vi "Main.vi"(11 "Module Admin":refnum<class "Delacor_lib_QMH_Module Admin.lvclass">) -> ()   [LabVIEW 2026, in "Launcher.lvlib"]
doc: "This template is based off of the Queued Message Handler design pattern and the Queued Message Handler project template that ships with LabVIEW.\n\nThe main difference is that the queue is private to this module and communication between modules is performed via Broadcast and Request events.\n\nRequest events are wrapped in public API methods and are handled in the Event Handling Loop (EHL) of this VI. Any module can register for Broadcast events sent by this module. The EHL generates messages based on user interface actions.\n\nThe Message Handling Loop (MHL) processes messages generated by the EHL, or by other messages. The messages are string values, so new messages can be added easily to the Message Cases case structure in the MHL. Each message cluster can also provide an optional value for Message Data, which is a variant that can be converted to whatever message-specific data is required.\n_____\nBased on DQMH Dev Tools: Project Template 7.1.2.1547."
uses:
  Launcher.lvlib
  <vilib>/Delacor/Delacor QMH/Libraries/Module Admin_class/Delacor_lib_QMH_Module Admin.lvclass
  <vilib>/Wovalab/Utilities/Helper Loop Periodic Timing/Late Execution Mode--enum.ctl
  <vilib>/Wovalab/Utilities/Helper Loop Periodic Timing/Helper Loop Periodic Timing.lvclass/Helper Loop Periodic Timing.ctl
  Module Data--cluster.ctl
  Mode.ctl
  ReplayMode.ctl
  RecordMode.ctl
  Capture detection loop data--cluster.ctl
  <vilib>/Delacor/Delacor QMH/Libraries/Message Queue_class/Delacor_lib_QMH_Message Queue.lvclass/Delacor_lib_QMH_Message Queue.ctl
  Stop Argument--cluster.ctl
  <vilib>/Delacor/Delacor QMH/Libraries/Module Admin_class/Delacor_lib_QMH_Module Admin.lvclass/Delacor_lib_QMH_Module Admin.ctl
  Set Captures Folder Argument--cluster.ctl
  Set Capture Detection Loop Timeout Argument--cluster.ctl
  Trigger Capture Detection Loop Argument--cluster.ctl
  Trigger Capture Detection Loop (Reply Payload)--cluster.ctl
  Set Application Mode Argument--cluster.ctl
  Set Run ID to Replay Argument--cluster.ctl
  <vilib>/Utility/miscctls.llb/LVPointTypeDef.ctl
  <vilib>/Delacor/Delacor QMH/Libraries/Message Queue_class/Delacor_lib_QMH_Enqueue Message (Single).vi
  <vilib>/Delacor/Delacor QMH/Libraries/Module Admin_class/Delacor_lib_QMH_Get External Launch.vi
  <vilib>/Wovalab/Utilities/Helper Loop Periodic Timing/Stop Helper Loop Internal.vi
  <vilib>/Wovalab/Utilities/Helper Loop Periodic Timing/U32 Max Value--constant.vi
  <vilib>/Wovalab/Utilities/Helper Loop Periodic Timing/Update Last Execution Time.vi
  <vilib>/Wovalab/Utilities/Helper Loop Periodic Timing/Loops Events AE.vi
  <vilib>/Wovalab/Utilities/Helper Loop Periodic Timing/Notify Monitoring Window.vi
  <vilib>/Wovalab/Utilities/Helper Loop Periodic Timing/Monitoring--global.vi
  <vilib>/Wovalab/Utilities/Helper Loop Periodic Timing/Helper Loop Periodic Timing.lvclass
  <vilib>/Delacor/Delacor QMH/Libraries/Message Queue_class/Delacor_lib_QMH_Message Queue.lvclass
  UserEventRecorder/UserEventRecorder.lvlib
  Core/Core.lvlib
  replay/Replay/src/Libraries/Replay/Replay.lvlib
panel:
  out "error out":errorcluster
  out "Status":string
  in  "Simulate MHL Error":bool
  in  "Simulate EHL Error":bool
  # "Other processes communicate with this Module via its Public API (wrappers for its Request Events).\n\nThis Module communicates with other processes via its Broadcast Events.\nAny process that wants to receive these messages can register for this module's Broadcast events."
  # "This template is for the DQMH framework. See the block diagram for more information on how to use this template."
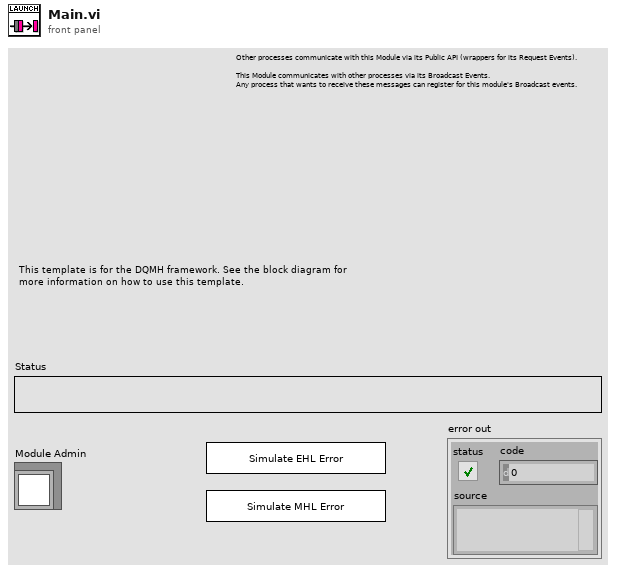
[diagram p1: front panel]
types:
  T1 = typedef "Wovalab_lib_Utilities.lvlib/Helper Loop Periodic Timing.lvclass/Late Execution Mode--enum.ctl" = enum16{"No change", "Process missed periods ignoring original phase", "Process missed periods maintaining original phase"}
  T2 = typedef "Launcher.lvlib/Broadcast Events--cluster.ctl" = cluster{"Module Did Init":refnum<user-event>, "Status Updated":refnum<user-event>, "Error Reported":refnum<user-event>, "Module Did Stop":refnum<user-event>, "Update Module Execution Status":refnum<user-event>, "Start Capture Detection Loop":refnum<user-event>, "Benchmark Started":refnum<user-event>, "Broadcast number of frames and run ID":refnum<user-event>}
  T3 = typedef "Launcher.lvlib/Request Events--cluster.ctl" = cluster{"Stop Module":refnum<user-event>, "Show Panel":refnum<user-event>, "Hide Panel":refnum<user-event>, "Get Module Execution Status":refnum<user-event>, "Show Diagram":refnum<user-event>, "Set Captures Folder":refnum<user-event>, "Set Capture Detection Loop Timeout":refnum<user-event>, "Trigger Capture Detection Loop":refnum<user-event>, "Set Application Mode":refnum<user-event>, "Application Mode":refnum<user-event>, "Set Run ID to Replay":refnum<user-event>, "Set Replay Run ID":refnum<user-event>}
  T4 = typedef "Capture detection loop data--cluster.ctl" = cluster{"Period":i32, "Reset":bool, "Iteration":i32, "Capture":path, "Mode":T5, "Replay Run ID":string, "Frame Number":u32, "Core Module ID":i32, "EventRecorderLaunched":bool, "Frame 0 relative seconds":dbl, "Record Run ID":string}
  T5 = typedef "Mode.ctl" = cluster{"Replay":T6, "Record":T7}
  T6 = typedef "ReplayMode.ctl" = enum16{"None", "User Events"}
  T7 = typedef "RecordMode.ctl" = enum16{"None", "User Events", "Benchmarks", "User Events and Benchmarks"}
  T8 = typedef "Launcher.lvlib/Module Data--cluster.ctl" = cluster{"Status":string, "Captures":path, "Capture Detection Loop Timeout":i32, "Mode":T5, "Replay Run ID":string, "Module Launched Timestamp":timestamp, "Record Run ID":i32, "Core Run ID":i32}
  T9 = enum32{"invalid lock state", "Not Locked", "Locked (No Password)", "Password-protected"}
  T10 = typedef "Launcher.lvlib/Stop Argument--cluster.ctl" = cluster{"Origin":string, "Exit via Stop Module Req?":bool, "Wait for Module to stop?":bool}
  T11 = typedef "Launcher.lvlib/Set Captures Folder Argument--cluster.ctl" = cluster{"Captures":path}
  T12 = typedef "Launcher.lvlib/Set Capture Detection Loop Timeout Argument--cluster.ctl" = cluster{"Timeout":i32}
  T13 = typedef "Launcher.lvlib/Trigger Capture Detection Loop Argument--cluster.ctl" = cluster{"Capture Detection Loop Timeout":i32, "Wait Notifier":refnum<notifier>, "wait for reply":bool}
  T14 = typedef "Launcher.lvlib/Set Application Mode Argument--cluster.ctl" = cluster{"Mode":T5}
  T15 = typedef "Launcher.lvlib/Set Run ID to Replay Argument--cluster.ctl" = cluster{"Run ID":string}
  T16 = typedef "LVPointTypeDef.ctl" = cluster{"Horizontal":i16, "Vertical":i16}
  T17 = enum32{"Invalid", "Standard", "Closed", "Hidden", "Minimized", "Maximized"}
  T18 = typedef "Launcher.lvlib/Trigger Capture Detection Loop (Reply Payload)--cluster.ctl" = cluster{"Module Initial Time Stamp":timestamp, "error":errorcluster}
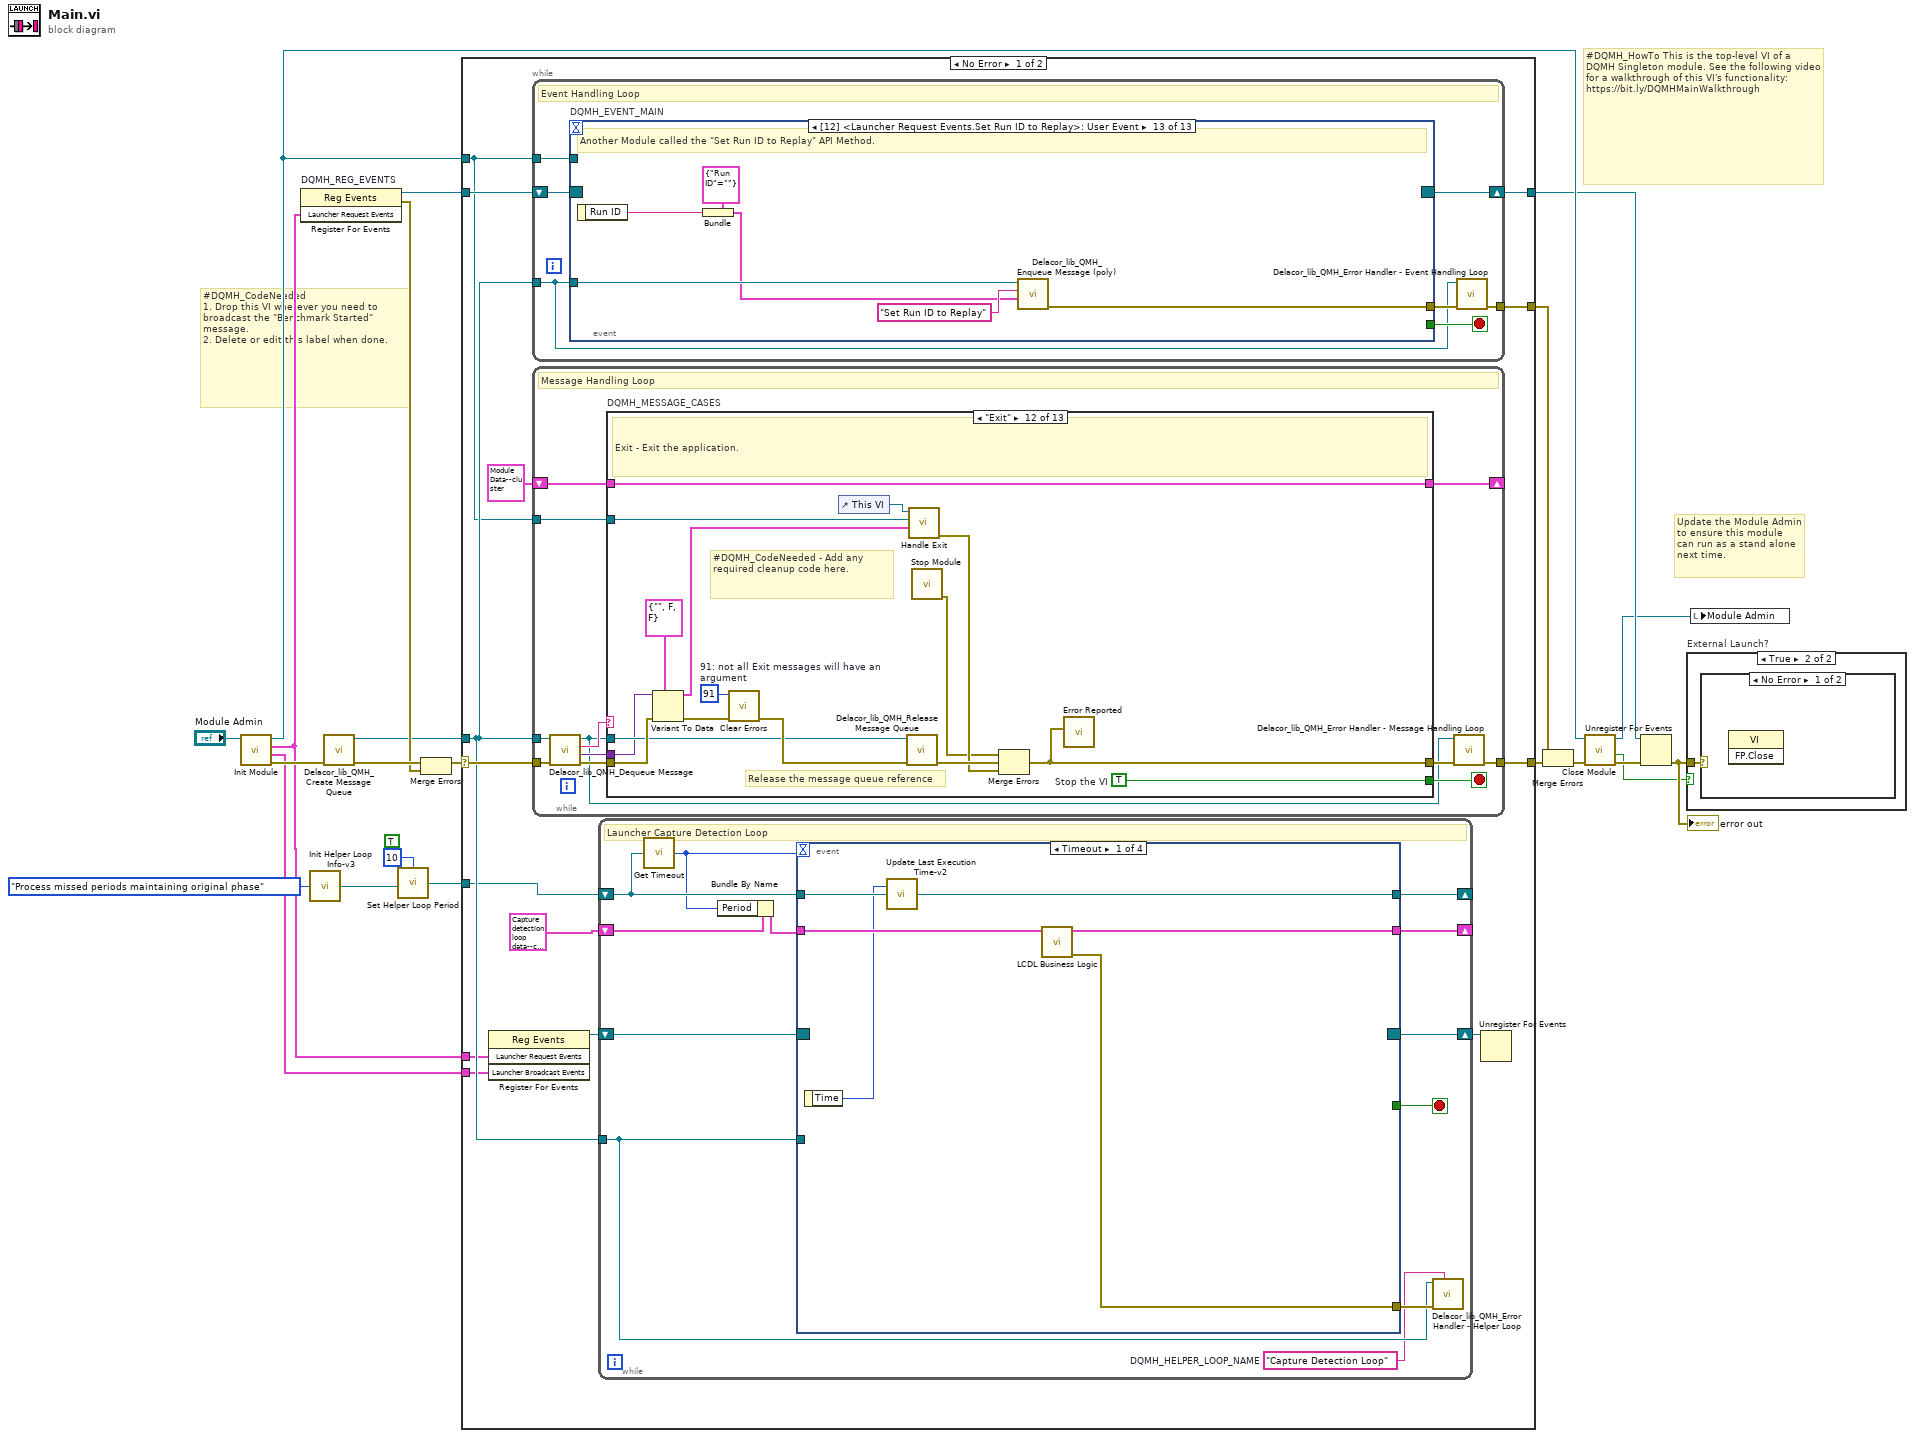
[diagram p0: block diagram]
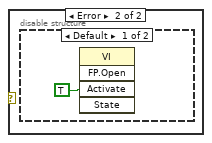
[diagram p3: hidden frame]
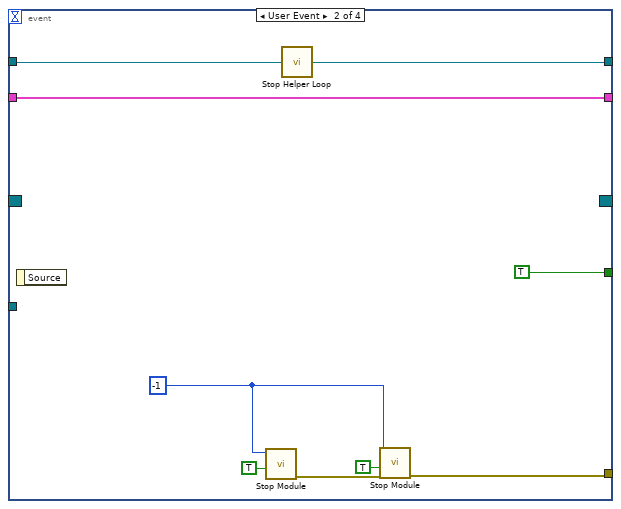
[diagram p5: hidden frame]
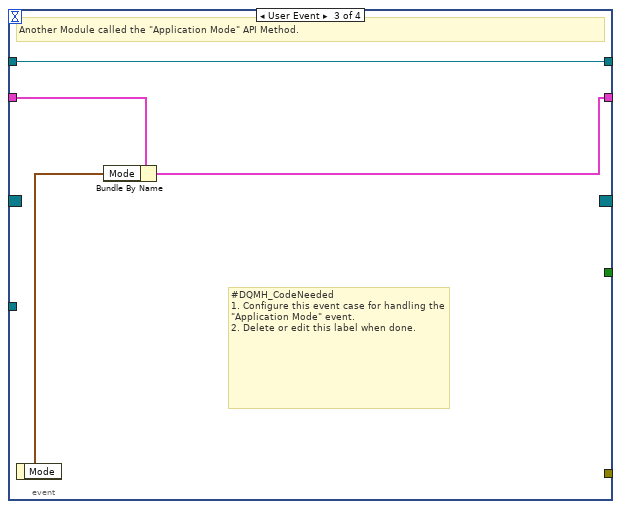
[diagram p6: hidden frame]
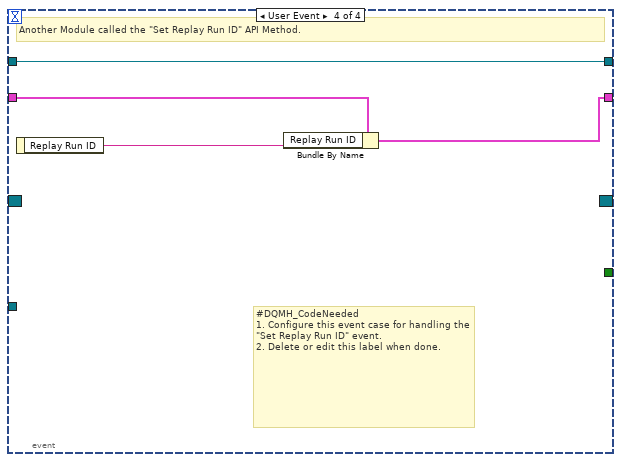
[diagram p7: hidden frame]
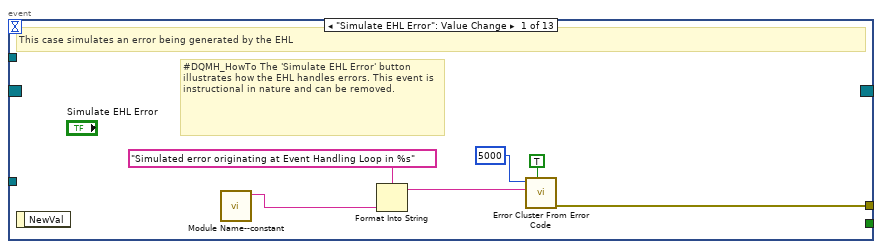
[diagram p8: hidden frame]
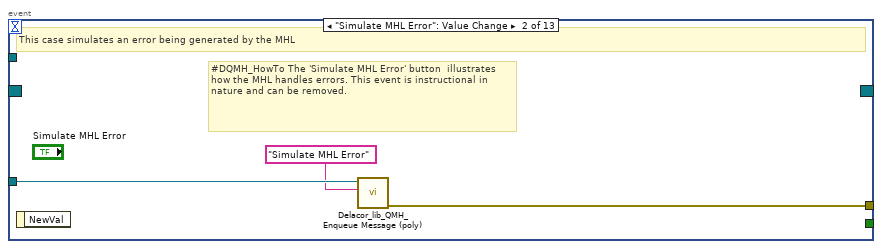
[diagram p9: hidden frame]
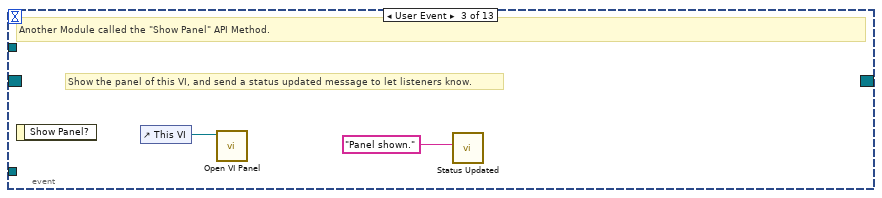
[diagram p10: hidden frame]
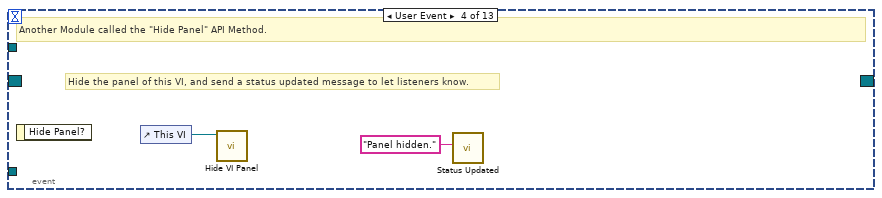
[diagram p11: hidden frame]
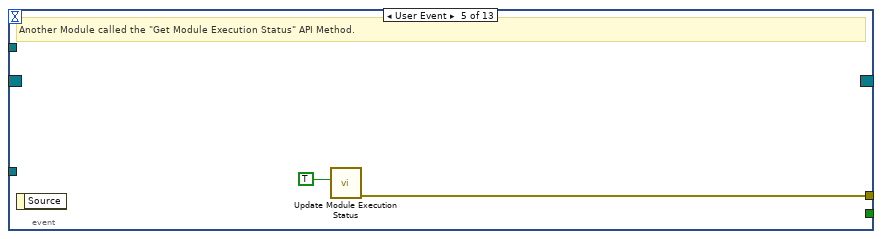
[diagram p12: hidden frame]
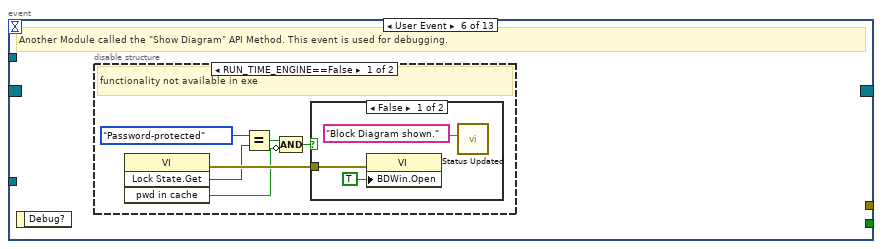
[diagram p13: hidden frame]
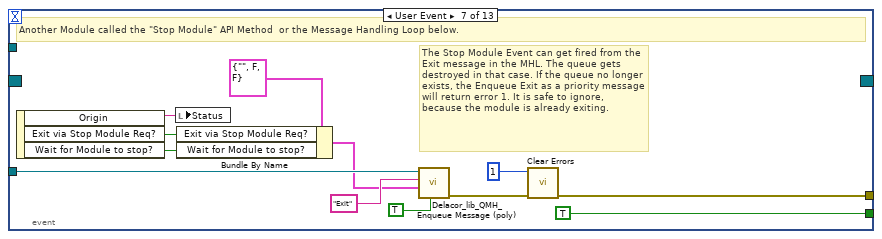
[diagram p16: hidden frame]
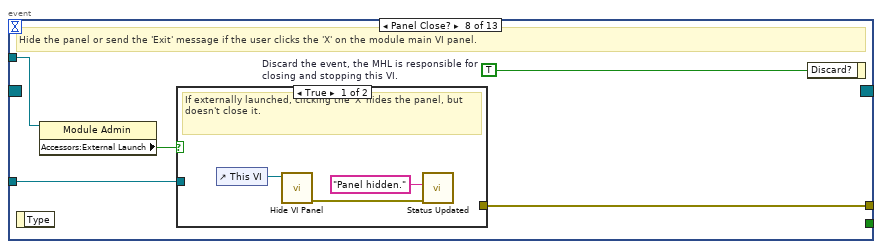
[diagram p17: hidden frame]
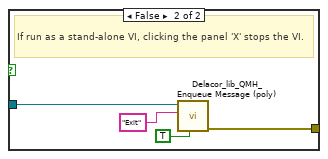
[diagram p18: hidden frame]
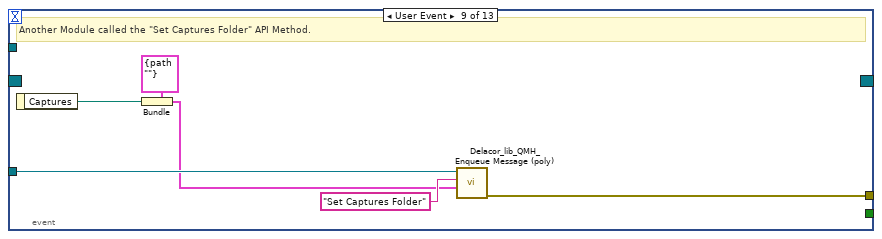
[diagram p19: hidden frame]
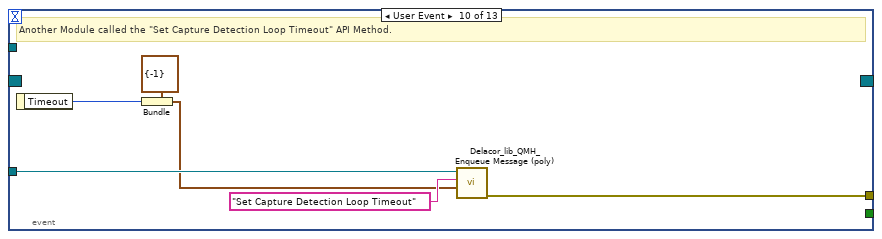
[diagram p20: hidden frame]
diagram:
  (unwired) TRUE ("Execute First Iteration ASAP (T)")
  # "#DQMH_CodeNeeded\n1. Drop this VI wherever you need to broadcast the \"Broadcast Latest Frame\" message.\n2. Delete or edit this label when done."
  # "#DQMH_CodeNeeded\n1. Drop this VI wherever you need to broadcast the \"Benchmark Started\" message.\n2. Delete or edit this label when done."
  # "#DQMH_HowTo This is the top-level VI of a DQMH Singleton module. See the following video for a walkthrough of this VI's functionality: https://bit.ly/DQMHMainWalkthrough"
  # "Update the Module Admin to ensure this module can run as a stand alone next time."
  n1 = call "Init Module.vi"("Singleton Module Admin in"="Module Admin") -> ("error out"=w21:errorcluster, "Launcher Broadcast Events"=w5:T2, "Launcher Request Events"=w6:T3, "Singleton Module Admin out"=w13:refnum<class "Delacor_lib_QMH_Module Admin.lvclass">)  [unwired: 7 in]
  n2 = register-events "DQMH_REG_EVENTS"(w6) -> (reference out=w11:refnum<event-registration>, error out=w14:errorcluster)  [unwired: 2 in]
  n3 = call <vilib>:"Init Helper Loop Info-v3.vi"("Late Execution Mode (Process missed periods ignoring original phase)"=Late_Execution_Mode--enum."Process missed periods maintaining original phase") -> ("Helper Loop Periodic Timing"=w3:refnum<class "Helper Loop Periodic Timing.lvclass">)  [unwired: 1 in]
  n4 = call <vilib>:"Delacor_lib_QMH_Create Message Queue.vi"("error in"=w21) -> ("error out"=w16:errorcluster, "Message Queue"=w10:refnum<class "Delacor_lib_QMH_Message Queue.lvclass">)  [unwired: 9 in]
  n5 = call <vilib>:"Set Helper Loop Period.vi"("Period (ms)"=10, "Helper Loop Periodic Timing in"=w3) -> ("Helper Loop Periodic Timing out"=w2:refnum<class "Helper Loop Periodic Timing.lvclass">)  [unwired: 13 in]
  n6 = Merge Errors(w16, w14) -> (w15:errorcluster)
  n7 = case shown="No Error" w15 {
    selector: w15 -> [w34 w321]
    tunnel: [w36 w320] -> w22
    tunnel: [w33 w319] -> w12
    tunnel: w11 -> [w31 w319]
    tunnel: w10 -> [w30 w314]
    tunnel: [w35 _] -> w19
    tunnel: w13 -> [w29 w315]
    tunnel: w6 -> [w28 _]
    tunnel: w5 -> [w25 _]
    tunnel: w2 -> [w23 _]
    frame No Error {
      n8 = register-events ("DQMH_HELPER_REGFOREVENTS")(w28, w25) -> (reference out=w26:refnum<event-registration>)  [unwired: 2 in, 1 out]
      n9 = while {
        tunnel: w30 -> [w72]
        shift-right: [w75] -> w33
        shift-left: w31 -> [w76]
        tunnel: [w77] -> w35
        tunnel: w29 -> [w73]
        stop <- w74 stop-if-true
        # "Event Handling Loop"
        n10 = event "DQMH_EVENT_MAIN" shown="[12] <Launcher Request Events.Set Run ID to Replay>: User Event" {
          selector: w76 -> [_ _ _ _ _ _ _ _ _ _ _ _ _]
          dyn-events: [_ _ _ _ _ _ _ _ _ _ _ _ _] -> w75
          timeout: _ -> [_ _ _ _ _ _ _ _ _ _ _ _ _]
          tunnel: [_ _ _ _ _ _ TRUE ("Discard?") _ _ _ _ _ _] -> w74
          tunnel: w72 -> [_ w86 _ _ _ _ w110 w117 w132 w138 w146 w152 w158]
          tunnel: [w84 w87 _ _ w93 _ w113 w119 w127 w133 w139 w147 w153] -> w78
          tunnel: w73 -> [_ _ _ _ _ _ _ w116 _ _ _ _ _]
          event "Simulate EHL Error": Value Change {
            # "#DQMH_HowTo The 'Simulate EHL Error' button  illustrates how the EHL handles errors. This event is instructional in nature and can be removed."
            # "This case simulates an error being generated by the EHL"
            n11 = event-data() -> ()  [unwired: 1 in, 1 out]
            n12 = call "Module Name--constant.vi"() -> ("Module Name"=w81:string)  [unwired: 11 in]
            n13 = Format Into String(format string="Simulated error originating at Event Handling Loop in %s", w81) -> (resulting string=w82:string)  [unwired: 2 in, 1 out]
            n14 = call <vilib>:"Error Cluster From Error Code.vi"("show call chain? (False)"=TRUE, "error message (\"\")"=w82, "error code (0)"=5000) -> ("error out"=w84:errorcluster)  [unwired: 6 in]
          }
          event "Simulate MHL Error": Value Change {
            # "#DQMH_HowTo The 'Simulate MHL Error' button  illustrates how the MHL handles errors. This event is instructional in nature and can be removed."
            # "This case simulates an error being generated by the MHL"
            n15 = event-data() -> ()  [unwired: 1 in, 1 out]
            n16 = call-poly <vilib>:"Delacor_lib_QMH_Enqueue Message (poly).vi"("Message"="Simulate MHL Error", "Message Queue in"=w86) -> ("error out"=w87:errorcluster)  [unwired: 8 in, 1 out]
          }
          event User Event {
            # "Show the panel of this VI, and send a status updated message to let listeners know."
            # "Another Module called the \"Show Panel\" API Method."
            n17 = event-data() -> ()  [unwired: 1 in, 1 out]
            n18 = control-ref of="This VI"() -> (w89:refnum<vi>)
            n19 = call "Open VI Panel.vi"("VI"=w89) -> ()  [unwired: 10 in, 1 out]
            n20 = call "Status Updated.vi"("Status"="Panel shown." ("format string")) -> ()  [unwired: 10 in, 1 out]
          }
          event User Event {
            # "Hide the panel of this VI, and send a status updated message to let listeners know."
            # "Another Module called the \"Hide Panel\" API Method."
            n21 = event-data() -> ()  [unwired: 1 in, 1 out]
            n22 = control-ref of="This VI"() -> (w91:refnum<vi>)
            n23 = call "Hide VI Panel.vi"("VI"=w91) -> ()  [unwired: 10 in, 1 out]
            n24 = call "Status Updated.vi"("Status"="Panel hidden." ("format string")) -> ()  [unwired: 10 in, 1 out]
          }
          event User Event {
            # "Another Module called the \"Get Module Execution Status\" API Method."
            n25 = event-data() -> ()  [unwired: 1 in, 1 out]
            n26 = call "Update Module Execution Status.vi"("Running?"=TRUE) -> ("error out"=w93:errorcluster)  [unwired: 10 in]
          }
          event User Event {
            # "Another Module called the \"Show Diagram\" API Method. This event is used for debugging."
            n27 = event-data() -> ()  [unwired: 1 in, 1 out]
            n28 = disable-structure shown="RUN_TIME_ENGINE==False" {
              frame condition #0 (active) {
                # "functionality not available in exe"
                n29 = invoke on="Invoke Node" class="VI" method="Lock State.Get"() -> (error out=w99:errorcluster, "Get Lock State"=w98:T9, "pwd in cache"=w95:bool)  [unwired: 4 in, 1 out]
                n30 = Equal?(x=T9."Password-protected", y=w98) -> (x = y?=w96:bool)
                n31 = Compound Arithmetic op=AND(w96, invert w95) -> (w94:bool)
                n32 = case shown="False" w94 {
                  tunnel: w99 -> [w102 _]
                  frame False {
                    n33 = property on="Property Node" class="VI"(error in=w102, "BDWin.Open"=TRUE ("Block Diagram Window:Open")) -> ()  [unwired: 1 in, 2 out]
                    n34 = call "Status Updated.vi"("Status"="Block Diagram shown." ("format string")) -> ()  [unwired: 10 in, 1 out]
                  }
                  frame True {
                    # "Password-protected VI, and the password is not in the cache. Do not show the diagram."
                  }
                }
              }
              frame condition #1 {
              }
            }
          }
          event User Event {
            # "The Stop Module Event can get fired from the Exit message in the MHL. The queue gets destroyed in that case. If the queue no longer exists, the Enqueue Exit as a priority message will return error 1. It is safe to ignore, because the module is already exiting."
            # "Another Module called the \"Stop Module\" API Method  or the Message Handling Loop below."
            n35 = event-data() -> ("Origin"=w109:string, "Exit via Stop Module Req?"=w105:bool, "Wait for Module to stop?"=w104:bool)  [unwired: 1 in]
            n36 = local write "Status"(w109) -> ()
            n37 = Bundle By Name(cluster=T10 {"Origin"="", "Exit via Stop Module Req?"=FALSE, "Wait for Module to stop?"=FALSE} ("Stop Argument"), "Exit via Stop Module Req?"=w105, "Wait for Module to stop?"=w104) -> (w103:T10)
            n38 = call-poly <vilib>:"Delacor_lib_QMH_Enqueue Message (poly).vi"("Priority Message? (F)"=TRUE, "Message Data"=w103, "Message"="Exit", "Message Queue in"=w110) -> ("error out"=w114:errorcluster)  [unwired: 6 in, 1 out]
            n39 = call <vilib>:"Clear Errors.vi"("error in (no error)"=w114, "specific error code to clear (0: all)"=1) -> ("error out"=w113:errorcluster)  [unwired: 4 in, 1 out]
          }
          event Panel Close? {
            w118 = TRUE  # Discard the event, the MHL is responsible for closing and stopping this VI.
            # "Hide the panel or send the 'Exit' message if the user clicks the 'X' on the module main VI panel."
            n40 = event-data() -> ()  [unwired: 1 in, 1 out]
            n41 = property on="Property Node" class="Module Admin"(reference=w116) -> ("Accessors:External Launch"=w115:bool)  [unwired: 1 in, 2 out]
            n42 = case shown="True" w115 {
              tunnel: w117 -> [_ w125]
              tunnel: [_ w126] -> w119
              frame True {
                # "If externally launched, clicking the 'X' hides the panel, but doesn't close it."
                n43 = control-ref of="This VI"() -> (w122:refnum<vi>)
                n44 = call "Hide VI Panel.vi"("VI"=w122) -> ("error out"=w120:errorcluster)  [unwired: 10 in]
                n45 = call "Status Updated.vi"("error in"=w120, "Status"="Panel hidden." ("format string")) -> ()  [unwired: 9 in, 1 out]
              }
              frame False {
                # "If run as a stand-alone VI, clicking the panel 'X' stops the VI."
                n46 = call-poly <vilib>:"Delacor_lib_QMH_Enqueue Message (poly).vi"("Priority Message? (F)"=TRUE, "Message"="Exit", "Message Queue in"=w125) -> ("error out"=w126:errorcluster)  [unwired: 7 in, 1 out]
              }
            }
            n47 = event-data ("Event Filter Node")("Discard?"=w118) -> ()  [unwired: 1 in, 1 out]
          }
          event User Event {
            # "Another Module called the \"Set Captures Folder\" API Method."
            n48 = event-data() -> ("Captures"=w128:path)  [unwired: 1 in]
            n49 = Bundle(cluster=T11 {"Captures"=path ""} ("Set Captures Folder Argument"), "Captures"=w128) -> (w129:T11)
            n50 = call-poly <vilib>:"Delacor_lib_QMH_Enqueue Message (poly).vi"("Message Data"=w129, "Message"="Set Captures Folder", "Message Queue in"=w132) -> ("error out"=w127:errorcluster)  [unwired: 7 in, 1 out]
          }
          event User Event {
            # "Another Module called the \"Set Capture Detection Loop Timeout\" API Method."
            n51 = event-data() -> ("Timeout"=w134:i32)  [unwired: 1 in]
            n52 = Bundle(cluster=T12 {"Timeout"=-1} ("Set Capture Detection Loop Timeout Argument"), "Timeout"=w134) -> (w135:T12)
            n53 = call-poly <vilib>:"Delacor_lib_QMH_Enqueue Message (poly).vi"("Message Data"=w135, "Message"="Set Capture Detection Loop Timeout", "Message Queue in"=w138) -> ("error out"=w133:errorcluster)  [unwired: 7 in, 1 out]
          }
          event User Event {
            # "Another Module called the \"Trigger Capture Detection Loop\" API Method."
            n54 = event-data() -> ("Capture Detection Loop Timeout"=w142:i32, "Wait Notifier"=w141:refnum<notifier>, "wait for reply"=w140:bool)  [unwired: 1 in]
            n55 = Bundle(cluster=T13 {"Capture Detection Loop Timeout"=-1, "Wait Notifier"=refnum, "wait for reply"=FALSE} ("Trigger Capture Detection Loop Argument"), "Capture Detection Loop Timeout"=w142, "Wait Notifier"=w141, "wait for reply"=w140) -> (w143:T13)
            n56 = call-poly <vilib>:"Delacor_lib_QMH_Enqueue Message (poly).vi"("Message Data"=w143, "Message"="Trigger Capture Detection Loop", "Message Queue in"=w146) -> ("error out"=w139:errorcluster)  [unwired: 7 in, 1 out]
          }
          event User Event {
            # "Another Module called the \"Set Application Mode\" API Method."
            n57 = event-data() -> ("Mode"=w148:T5)  [unwired: 1 in]
            n58 = Bundle(cluster=T14 {"Mode"={"Replay"=enum."None", "Record"=enum."None"}} ("Set Application Mode Argument"), "Mode"=w148) -> (w149:T14)
            n59 = call-poly <vilib>:"Delacor_lib_QMH_Enqueue Message (poly).vi"("Message Data"=w149, "Message"="Set Application Mode", "Message Queue in"=w152) -> ("error out"=w147:errorcluster)  [unwired: 7 in, 1 out]
          }
          event User Event {
            # "Another Module called the \"Set Run ID to Replay\" API Method."
            n60 = event-data() -> ("Run ID"=w154:string)  [unwired: 1 in]
            n61 = Bundle(cluster=T15 {"Run ID"=""} ("Set Run ID to Replay Argument"), "Run ID"=w154) -> (w155:T15)
            n62 = call-poly <vilib>:"Delacor_lib_QMH_Enqueue Message (poly).vi"("Message Data"=w155, "Message"="Set Run ID to Replay", "Message Queue in"=w158) -> ("error out"=w153:errorcluster)  [unwired: 7 in, 1 out]
          }
        }
        n63 = call-dynamic "Delacor_lib_QMH_Error Handler - Event Handling Loop.vi"("error in"=w78, "Message Queue in"=w72) -> ("dup error in"=w77:errorcluster)  [unwired: 8 in, 1 out]
      }
      n64 = while {
        tunnel: w30 -> [w159]
        shift-right: [w167] -> _
        shift-left: T8 {"Status"="", "Captures"=path "", "Capture Detection Loop Timeout"=0, "Mode"={"Replay"=enum."None", "Record"=enum."None"}, "Replay Run ID"="", "Module Launched Timestamp"=timestamp(0 s since 1904-01-01), "Record Run ID"=0, "Core Run ID"=0} ("Data Cluster") -> [w168]
        tunnel: w34 -> [w170]
        tunnel: [w162] -> w36
        tunnel: w29 -> [w163]
        stop <- w166 stop-if-true
        # "Message Handling Loop"
        n65 = call-dynamic "Delacor_lib_QMH_Dequeue Message.vi"("error in"=w170, "Message Queue in"=w159) -> ("error out"=w169:errorcluster, "Message Data"=w164:variant, "Message"=w165:string, "Message Queue out"=w160:refnum<class "Delacor_lib_QMH_Message Queue.lvclass">)  [unwired: 6 in]
        n66 = case "DQMH_MESSAGE_CASES" shown="\"Exit\"" w165 {
          selector: w165 -> [_ _ _ _ _ _ _ _ _ _ _ _ w309]
          tunnel: w160 -> [_ _ _ _ _ _ _ _ _ _ w274 w297 _]
          tunnel: w169 -> [w202 w206 w217 w226 w238 w248 w256 w259 w261 w270 w281 w303 w312]
          tunnel: [w201 w206 w211 w221 w229 w247 w255 w258 w261 w269 w277 w298 w313] -> w161
          tunnel: w168 -> [w192 w205 w209 w220 w237 w243 w251 w257 w260 w267 w276 w296 w310]
          tunnel: [w191 w205 w213 w220 w237 w242 w250 w257 w260 w267 w276 w296 w310] -> w167
          tunnel: [_ _ _ _ _ _ _ _ _ _ _ w295 _] -> w166
          tunnel: w164 -> [_ _ w216 w225 w236 w246 w254 _ _ _ w275 w294 _]
          tunnel: w163 -> [w193 _ _ _ _ _ _ _ _ _ w273 w289 _]
          frame "Initialize" {
            w187 = "Initial Message" ("Initial Message")
            # "#DQMH_CodeNeeded - Initialize the appearance of the front panel."
            # "#DQMH_CodeNeeded - Initialize your state data here."
            # "Initialize - Any operation that needs to be done before the module can receive messages. Synchronize Caller Events.vi will inform Start Module.vi that the module has launched and is ready to receive messages. Module Did Init.vi will broadcast that the module initialized."
            n67 = call "Synchronize Caller Events.vi"("error in"=w202, "Singleton Module Admin in"=w193) -> ("error out"=w184:errorcluster, "Singleton Module Admin out"=w188:refnum<class "Delacor_lib_QMH_Module Admin.lvclass">)  [unwired: 8 in]
            n68 = property on="Pane" class="Pane"("Origin"=T16 {"Horizontal"=0, "Vertical"=0}) -> ()  [unwired: 2 in, 2 out]
            n69 = property on="Property Node" class="Module Admin"(reference=w188) -> ("Accessors:External Launch"=w197:bool)  [unwired: 1 in, 2 out]
            n70 = call "Module Name--constant.vi"() -> ("Module Name"=w200:string)  [unwired: 11 in]
            n71 = property on="Property Node" class="VI"("Front Panel.Title"=w200) -> (reference out=w199:refnum<vi>, error out=w204:errorcluster)  [unwired: 2 in]
            n72 = Select(t=T17."Hidden" ("State"), s=w197, f=T17."Standard" ("State")) -> (s? t:f=w194:T17)
            n73 = invoke on="Invoke Node" class="VI" method="FP.Open"(reference=w199, error in=w204, "State"=w194) -> (reference out=w198:refnum<vi>, error out=w203:errorcluster)  [unwired: 2 in, 3 out]
            n74 = call "Start Module.vi"("error in"=w184) -> ("error out"=w183:errorcluster, "Wait for Event Sync?"=w181:bool, "Module ID"=w182:i32)  [unwired: 6 in, 2 out]
            n75 = invoke on="Invoke Node" class="VI" method="FP.Center"(reference=w198, error in=w203) -> ()  [unwired: 1 in, 3 out]
            n76 = call "Synchronize Module Events.vi"("error in"=w183, "Wait for Event Sync?"=w181, "Module ID in"=w182) -> ("error out"=w179:errorcluster, "Module ID out"=w180:i32)  [unwired: 7 in]
            n77 = Get Date/Time In Seconds() -> (seconds since 1Jan1904=w185:timestamp)
            n78 = call "Start Module.vi"("error in"=w179) -> ("error out"=w178:errorcluster, "Wait for Event Sync?"=w176:bool, "Module ID"=w177:i32)  [unwired: 6 in, 2 out]
            n79 = call "Synchronize Module Events.vi"("error in"=w178, "Wait for Event Sync?"=w176, "Module ID in"=w177) -> ("error out"=w174:errorcluster, "Module ID out"=w175:i32)  [unwired: 7 in]
            n80 = call "Start Module.vi"("error in"=w174) -> ("error out"=w173:errorcluster, "Wait for Event Sync?"=w171:bool)  [unwired: 6 in, 3 out]
            n81 = call "Synchronize Module Events.vi"("error in"=w173, "Wait for Event Sync?"=w171) -> ("error out"=w172:errorcluster)  [unwired: 9 in]
            n82 = Bundle By Name(cluster=w192, "Module Launched Timestamp"=w185, "Status"=w187, "Record Run ID"=w180, "Core Run ID"=w175) -> (w191:T8)
            n83 = call "Module Name--constant.vi"() -> ("Module Name"=w189:string)  [unwired: 11 in]
            n84 = call "Module Did Init.vi"("error in"=w172, "Initialized?"=TRUE, "Origin"=w189) -> ("error out"=w201:errorcluster)  [unwired: 8 in]
            "Status" <- w187
          }
          frame "---Module Specific---" {
            # "Separator -- The following cases handle messages specific to this Module."
          }
          frame "Set Captures Folder" {
            n85 = Variant To Data(error in=w217, type=T11 {"Captures"=path ""} ("Set Captures Folder Argument"), Variant=w216) -> (data=w214:T11, error out=w212:errorcluster)
            n86 = Unbundle By Name(w214) -> ("Captures"=w208:path)
            n87 = Unbundle By Name(w209) -> ("Capture Detection Loop Timeout"=w210:i32, "Module Launched Timestamp"=w207:timestamp)
            n88 = Bundle By Name(cluster=w209, "Captures"=w208) -> (w213:T8)
            n89 = call "Start Capture Detection Loop.vi"("error in"=w212, "Module Launched Timestamp"=w207, "Period"=w210) -> ("error out"=w211:errorcluster)  [unwired: 8 in]
          }
          frame "Set Capture Detection Loop Timeout" {
            # "#DQMH_CodeNeeded\n1. Configure this Message Case for handling the \"Set Capture Detection Loop Timeout\" message.\n2. Delete or edit this label when done."
            n90 = Variant To Data(error in=w226, type=T12 {"Timeout"=-1} ("Set Capture Detection Loop Timeout Argument"), Variant=w225) -> (data=w223:T12, error out=w222:errorcluster)
            n91 = Unbundle By Name(w223) -> ()  [unwired: 1 out]
            n92 = Unbundle By Name(w220) -> ("Module Launched Timestamp"=w219:timestamp)
            n93 = call "Start Capture Detection Loop.vi"("error in"=w222, "Module Launched Timestamp"=w219, "Period"=1) -> ("error out"=w221:errorcluster)  [unwired: 8 in]
          }
          frame "Trigger Capture Detection Loop" {
            (unwired) 0  # Capture Detection Loop Timeout
            # "#DQMH_CodeNeeded\n1. Configure this Message Case for handling the \"Trigger Capture Detection Loop\" message.\n2. Wire any error that occurs to the \"error\" terminal.\n3. Delete or edit this label when done."
            n94 = Variant To Data(error in=w238, type=T13 {"Capture Detection Loop Timeout"=-1, "Wait Notifier"=refnum, "wait for reply"=FALSE} ("Trigger Capture Detection Loop Argument"), Variant=w236) -> (data=w234:T13, error out=w227:errorcluster)
            n95 = Unbundle By Name(w234) -> ("Wait Notifier"=w233:refnum<notifier>, "wait for reply"=w232:bool)  [unwired: 1 out]
            n96 = Get Date/Time In Seconds() -> (seconds since 1Jan1904=w228:timestamp)
            n97 = Bundle By Name(cluster=T18 {"Module Initial Time Stamp"=timestamp(0 s since 1904-01-01), "error"={"status"=FALSE, "code"=0, "source"=""}} ("Trigger Capture Detection Loop (Reply Payload)"), "Module Initial Time Stamp"=w228, "error"=w227) -> (w231:T18)
            n98 = Merge Errors(w227) -> (w229:errorcluster)
            n99 = case "DQMH_FIRE_NOTIFIER" shown="True" w232 {
              tunnel: w233 -> [_ w240]
              tunnel: w231 -> [_ w239]
              frame False {
              }
              frame True {
                n100 = Send Notification(notification=w239, notifier=w240) -> ()  [unwired: 1 in, 2 out]
              }
            }
          }
          frame "Set Application Mode" {
            n101 = Variant To Data(error in=w248, type=T14 {"Mode"={"Replay"=enum."None", "Record"=enum."None"}} ("Set Application Mode Argument"), Variant=w246) -> (data=w244:T14, error out=w247:errorcluster)
            n102 = Unbundle By Name(w244) -> ("Mode"=w241:T5)
            n103 = Bundle By Name(cluster=w243, "Mode"=w241) -> (w242:T8)
          }
          frame "Set Run ID to Replay" {
            # "#DQMH_CodeNeeded\n1. Configure this Message Case for handling the \"Set Run ID to Replay\" message.\n2. Delete or edit this label when done."
            n104 = Variant To Data(error in=w256, type=T15 {"Run ID"=""} ("Set Run ID to Replay Argument"), Variant=w254) -> (data=w252:T15, error out=w255:errorcluster)
            n105 = Unbundle By Name(w252) -> ("Run ID"=w249:string)
            n106 = Bundle By Name(cluster=w251, "Replay Run ID"=w249) -> (w250:T8)
          }
          frame "---Copy This Frame---" {
            # "Duplicate this frame when creating new messages.  Change this comment in the duplicated frame to describe this message."
            n107 = Merge Errors(w259) -> (w258:errorcluster)
          }
          frame "---Exit and Error Handling---" {
            # "Separator - The following cases handle errors and exit messages."
          }
          frame "Simulate MHL Error" {
            # "#DQMH_HowTo The 'Simulate MHL Error' button  illustrates how the MHL handles errors. This event is instructional in nature and can be removed."
            # "Simulate an error occurring at the MHL"
            n108 = call "Module Name--constant.vi"() -> ("Module Name"=w263:string)  [unwired: 11 in]
            n109 = Format Into String(format string="Simulated error originating at Message Handling Loop in %s", w263) -> (resulting string=w264:string)  [unwired: 2 in, 1 out]
            n110 = call <vilib>:"Error Cluster From Error Code.vi"("show call chain? (False)"=TRUE, "error message (\"\")"=w264, "error code (0)"=5001) -> ("error out"=w268:errorcluster)  [unwired: 6 in]
            n111 = Merge Errors(w270, w268) -> (w269:errorcluster)
          }
          frame "Error" {
            # "#DQMH_CodeRecommended - If the module is running in standalone mode (External Launch = FALSE), this code will pop up an error dialog and call the 'Exit' message if an error occurs. Add more fine-grained error management here."
            # "Error - Check the error message data and respond accordingly. This message is sent by the \"Error Handler\" VIs at the end of each loop in this application."
            n112 = property on="Property Node" class="Module Admin"(reference=w273) -> ("Accessors:External Launch"=w272:bool)  [unwired: 1 in, 2 out]
            n113 = Variant To Data(error in=w281, type=errorcluster {"status"=FALSE, "code"=0, "source"=""} ("error constant"), Variant=w275) -> (data=w271:errorcluster, error out=w279:errorcluster)
            n114 = local write "error out"(w271) -> ()
            n115 = call "Error Reported.vi"("Error"=w271) -> ()  [unwired: 10 in, 1 out]
            n116 = case shown="False" w272 {
              tunnel: [w286 _] -> w278
              tunnel: w274 -> [w284 _]
              tunnel: w271 -> [w285 _]
              frame False {
                n117 = disable-structure shown="Default" {
                  disable-tunnel: w285 -> [w287 _]
                  frame condition #0 (active) {
                    # "If the module is running standalone, then pop up an error dialog and call the \"Exit\" message."
                    n118 = call <vilib>:"Simple Error Handler.vi"("error in (no error)"=w287) -> ()  [unwired: 4 in, 5 out]
                  }
                  frame condition #1 {
                    # "To prevent the Simple Error Handler VI from being loaded (e.g. when deploying to a Real-Time target), add the Conditional Disable Symbol \"DQMH_Disable_SEH\" to your project and set it to TRUE."
                  }
                }
                n119 = call-poly <vilib>:"Delacor_lib_QMH_Enqueue Message (poly).vi"("Priority Message? (F)"=TRUE, "Message"="Exit", "Message Queue in"=w284) -> ("error out"=w286:errorcluster)  [unwired: 7 in, 1 out]
              }
              frame True {
                # "If the module was launched externally, calling the Error Reported broadcast VI is the only action performed by the \"Error\" message. The module's caller can then process the error appropriately."
              }
            }
            n120 = Merge Errors(w279, w278) -> (w277:errorcluster)
          }
          frame "Exit" {
            w293 = 91  # 91: not all Exit messages will have an argument
            w295 = TRUE  # Stop the VI
            # "Release the message queue reference"
            # "#DQMH_CodeNeeded - Add any required cleanup code here."
            # "Exit - Exit the application."
            n121 = Variant To Data(error in=w303, type=T10 {"Origin"="", "Exit via Stop Module Req?"=FALSE, "Wait for Module to stop?"=FALSE} ("Stop Argument"), Variant=w294) -> (data=w291:T10, error out=w300:errorcluster)
            n122 = call <vilib>:"Clear Errors.vi"("error in (no error)"=w300, "specific error code to clear (0: all)"=w293) -> ("error out"=w302:errorcluster)  [unwired: 4 in, 1 out]
            n123 = control-ref of="This VI"() -> (w290:refnum<vi>)
            n124 = call-dynamic "Delacor_lib_QMH_Release Message Queue.vi"("error in"=w302, "Message Queue"=w297) -> ("error out"=w301:errorcluster)  [unwired: 9 in]
            n125 = call "Handle Exit.vi"("Stop Argument"=w291, "Admin in"=w289, "VI reference"=w290) -> ("error out"=w299:errorcluster)  [unwired: 7 in, 1 out]
            n126 = call "Stop Module.vi"() -> ("error out"=w288:errorcluster)  [unwired: 11 in]
            n127 = Merge Errors(w288, w301, w299) -> (w298:errorcluster)
            n128 = call "Error Reported.vi"("Error"=w298) -> ()  [unwired: 10 in, 1 out]
          }
          frame Default {
            # "'Default' case only runs if there is a message that isn't defined in any of the other cases.  Output a programming error."
            n129 = call "Module Name--constant.vi"() -> ("Module Name"=w308:string)  [unwired: 11 in]
            n130 = Format Into String(format string="The invalid message string \"%s\" was received in the Message Handling Loop for module \"%s\".", w309, w308) -> (resulting string=w304:string)  [unwired: 2 in, 1 out]
            n131 = call <vilib>:"Error Cluster From Error Code.vi"("show call chain? (False)"=TRUE, "error message (\"\")"=w304, "error code (0)"=1) -> ("error out"=w311:errorcluster)  [unwired: 6 in]
            n132 = Merge Errors(w312, w311) -> (w313:errorcluster)
          }
        }
        n133 = call-dynamic "Delacor_lib_QMH_Error Handler - Message Handling Loop.vi"("error in"=w161, "Message Queue in"=w160) -> ("dup error in"=w162:errorcluster)  [unwired: 8 in, 1 out]
      }
      n134 = while "DQMH_HELPER_LOOP" {
        shift-right: [w47] -> w27
        shift-left: w26 -> [w48]
        tunnel: w30 -> [w44]
        shift-right: [w42] -> _
        shift-left: T4 {"Period"=84, "Reset"=TRUE, "Iteration"=0, "Capture"=path "", "Mode"={"Replay"=enum."None", "Record"=enum."None"}, "Replay Run ID"="", "Frame Number"=0, "Core Module ID"=0, "EventRecorderLaunched"=FALSE, "Frame 0 relative seconds"=0.0, "Record Run ID"=""} ("CaptureDetectionLoopData") -> [w41]
        shift-right: [w37] -> _
        shift-left: w23 -> [w39]
        stop <- w46 stop-if-true
        w43 = "Capture Detection Loop"  # DQMH_HELPER_LOOP_NAME
        # "Launcher Capture Detection Loop"
        n135 = call <vilib>:"Get Timeout.vi"("Helper Loop Periodic Timing"=w39) -> ("Timeout (ms)"=w38:i32)  [unwired: 12 in, 2 out]
        n136 = Bundle By Name(cluster=w41, "Period"=w38) -> (w40:T4)
        n137 = event "DQMH_HELPER_EVENT_STRUCTURE" shown="[0] Timeout" {
          selector: w48 -> [_ _ _ _]
          dyn-events: [_ _ _ _] -> w47
          timeout: w38 -> [_ _ _ _]
          tunnel: [_ TRUE _ _] -> w46
          tunnel: [w52 w56 _ _] -> w45
          tunnel: w44 -> [_ _ _ _]
          tunnel: w40 -> [w54 w62 w67 w71]
          tunnel: [w53 w62 w65 w70] -> w42
          tunnel: w39 -> [w51 w61 w64 w68]
          tunnel: [w49 w60 w64 w68] -> w37
          event Timeout {
            n138 = event-data() -> ("Time"=w50:u32)  [unwired: 1 in]
            n139 = call <vilib>:"Update Last Execution Time-v2.vi"("Time"=w50, "Helper Loop Periodic Timing in"=w51) -> ("Helper Loop Periodic Timing out"=w49:refnum<class "Helper Loop Periodic Timing.lvclass">)  [unwired: 12 in, 1 out]
            n140 = call "LCDL Business Logic.vi"("CaptureDetectionLoopDataIn"=w54) -> ("error out"=w52:errorcluster, "CaptureDetectionLoopDataOut"=w53:T4)  [unwired: 8 in, 1 out]
          }
          event User Event {
            w55 = -1 ("Module ID")
            n141 = event-data() -> ()  [unwired: 1 in, 1 out]
            n142 = call "Stop Module.vi"("Wait for Module to stop? (F)"=TRUE, "Module ID"=w55) -> ("error out"=w57:errorcluster)  [unwired: 9 in]
            n143 = call <vilib>:"Stop Helper Loop.vi"("Helper Loop Periodic Timing in"=w61) -> ("Helper Loop Periodic Timing out"=w60:refnum<class "Helper Loop Periodic Timing.lvclass">)
            n144 = call "Stop Module.vi"("error in"=w57, "Wait for Module to stop? (F)"=TRUE, "Module ID"=w55) -> ("error out"=w56:errorcluster)  [unwired: 8 in]
          }
          event User Event {
            # "#DQMH_CodeNeeded\n1. Configure this event case for handling the \"Application Mode\" event.\n2. Delete or edit this label when done."
            # "Another Module called the \"Application Mode\" API Method."
            n145 = event-data() -> ("Mode"=w66:T5)  [unwired: 1 in]
            n146 = Bundle By Name(cluster=w67, "Mode"=w66) -> (w65:T4)
          }
          event User Event {
            # "#DQMH_CodeNeeded\n1. Configure this event case for handling the \"Set Replay Run ID\" event.\n2. Delete or edit this label when done."
            # "Another Module called the \"Set Replay Run ID\" API Method."
            n147 = event-data() -> ("Replay Run ID"=w69:string)  [unwired: 1 in]
            n148 = Bundle By Name(cluster=w71, "Replay Run ID"=w69) -> (w70:T4)
          }
        }
        n149 = call-dynamic "Delacor_lib_QMH_Error Handler - Helper Loop.vi"("Error Debug"=w43, "error in"=w45, "Message Queue in"=w44) -> ()  [unwired: 7 in, 2 out]
      }
      n150 = Unregister For Events(event registration refnum=w27) -> ()  [unwired: 1 in, 1 out]
    }
    frame Error {
      # "Synchronize Caller Events.vi will inform Start Module.vi that the module has launched and will let the code calling Start Module.vi register for broadcasts and would permit the caller receive the broadcast that an error occurred at launch time."
      n151 = call-dynamic "Delacor_lib_QMH_Release Message Queue.vi"("error in"=w321, "Message Queue"=w314) -> ("error out"=w320:errorcluster)  [unwired: 9 in]
      n152 = call "Synchronize Caller Events.vi"("Singleton Module Admin in"=w315) -> ("error out"=w322:errorcluster)  [unwired: 9 in, 1 out]
      n153 = call "Module Name--constant.vi"() -> ("Module Name"=w318:string)  [unwired: 11 in]
      n154 = Format Into String(format string="An error occurred during initialization. %s is no longer running.", w318) -> (resulting string=w316:string)  [unwired: 2 in, 1 out]
      n155 = Merge Errors(w320, w322) -> (w323:errorcluster)
      n156 = call "Error Reported.vi"("Additional Information"=w316, "Error"=w323) -> ()  [unwired: 9 in, 1 out]
    }
  }
  n157 = Merge Errors(w19, w22) -> (w18:errorcluster)
  n158 = call "Close Module.vi"("error in"=w18, "Module Admin in"=w13) -> ("error out"=w20:errorcluster, "External Launch"=w7:bool, "Module Admin out"=w8:refnum<class "Delacor_lib_QMH_Module Admin.lvclass">)  [unwired: 7 in]
  n159 = Unregister For Events(event registration refnum=w12, error in=w20) -> (error out=w17:errorcluster)
  "error out" <- w17
  n160 = case "External Launch?" shown="True" w7 {
    tunnel: w17 -> [_ w324]
    frame False {
    }
    frame True {
      n161 = case shown="No Error" w324 {
        frame No Error {
          n162 = invoke on="Invoke Node" class="VI" method="FP.Close"() -> ()  [unwired: 3 in, 3 out]
        }
        frame Error {
          n163 = disable-structure shown="Default" {
            frame condition #0 (active) {
              n164 = invoke class="VI" method="FP.Open"("Activate"=TRUE ("Activate?")) -> ()  [unwired: 4 in, 5 out]
            }
            frame condition #1 {
              # "Don't show panel on error if running inside a built EXE."
            }
          }
        }
      }
    }
  }
  n165 = local write "Module Admin"(w8) -> ()
